vi "CE Client - CalcExpress.vi"(6 "error in":errorcluster, 8 "expression":string, 9 "CE session":T3={"VI refnum"=refnum, "VC Handle"=-1}) -> (0 "error out":errorcluster, 2 "values out":T2={"type"=enum."DBL Number", "dbl"=0.0, "cdb"=0.0+0.0i, "str"="", "1d dbl"=[], "1d cdb"=[], "1d str"=[], "2d dbl"=[], "2d cdb"=[], "2d str"=[]} {"2d cdb" format="%.2f"; "2d dbl" format="%.2f"; "1d cdb" format="%.2f"; "1d dbl" format="%.2f"; "cdb" format="%.2f"; "dbl" format="%.2f"}, 3 "dup CE session":T3={"VI refnum"=refnum, "VC Handle"=-1})   [LabVIEW 2021]
doc: "::: CalcExpress Toolkit :::\nCopyright (c) 2000-2026 Konstantin Shifershteyn. All rights reserved."
uses:
  CE Session.ctl
  vi.lib/addons/CalcExpress/cetypes.llb/VarMan Variable Context Handle.ctl
  vi.lib/addons/CalcExpress/cetypes.llb/CalcExpress Data Type.ctl
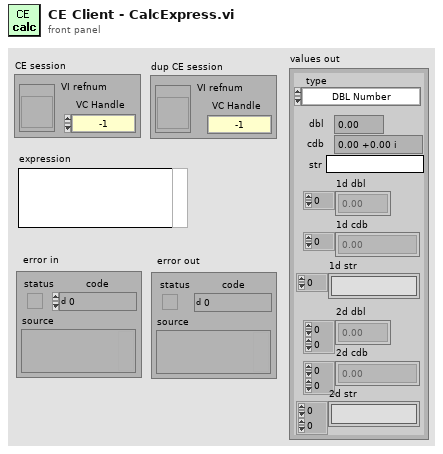
[diagram p1: front panel]
types:
  T1 = typedef "CalcExpress Data Type.ctl" = enum32{"String", "DBL Number", "identifier", "1D Array of DBL", "2D Array of DBL", "CDB Number", "1D Array of CDB", "2D Array of CDB", "1D Array of String", "2D Array of String", "Unknown data type"}
  T2 = cluster{"type":T1, "dbl":dbl, "cdb":cdb, "str":string, "1d dbl":dbl[], "1d cdb":cdb[], "1d str":string[], "2d dbl":dbl[][], "2d cdb":cdb[][], "2d str":string[][]}
  T3 = typedef "CE Session.ctl" = cluster{"VI refnum":refnum<vi>, "VC Handle":T4}
  T4 = typedef "VarMan Variable Context Handle.ctl" = i32
  T5 = enum16{"open session", "close session", "CalcExpress", "VarMan", "VarMan (low level)"}
  T6 = cluster{"type":enum32{"String", "DBL Number", "identifier", "1D Array of DBL", "2D Array of DBL", "CDB Number", "1D Array of CDB", "2D Array of CDB", "1D Array of String", "2D Array of String", "Unknown data type"}, "dbl":dbl, "cdb":cdb, "str":string, "1d dbl":dbl[], "1d cdb":cdb[], "1d str":string[], "2d dbl":dbl[][], "2d cdb":cdb[][], "2d str":string[][]}
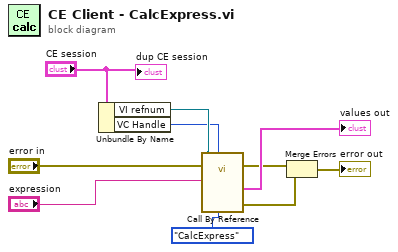
[diagram p0: block diagram]
diagram:
  n1 = Unbundle By Name("CE session") -> ("VI refnum"=w10:refnum<vi>, "VC Handle"=w9:T4)
  n2 = call-by-ref "?"(reference=w10, error in="error in", "exec"=T5."CalcExpress", "VC Handle"=w9, "expression/name"="expression") -> (error out=w1:errorcluster, "error out"=w3:errorcluster, "values out"=→"values out":T6)  [unwired: 6 in, 2 out]
  n3 = Merge Errors(w1, w3) -> (→"error out":errorcluster)
  "dup CE session" <- "CE session"
